vi "Complete Modern MCP Result.vi"(6 "parameters":string[][](array[string]), 7 "id in":i32, 8 "error in":errorcluster, 9 "input requests":string, 10 "handler response":string, 11 "MCP Request Metadata":T1) -> (0 "error out":errorcluster, 2 "status code":u16, 3 "response":string)   [LabVIEW 2020, in "MCP Server.lvlib"]
doc: "Turns what the request handler answered into the HTTP response body and status of a request that was not refused.\n\nLEGACY requests: the handler's answer is returned unchanged.\n\nMODERN requests (MCP 2026-07-28):\n- server/discover is answered here (supportedVersions = all versions, capabilities and serverInfo as initialize reports them, and the cache hints of Cache Hints.vi).\n- A tools/call for which a tool registered questions is answered with {\"resultType\":\"input_required\",\"inputRequests\":{...}} instead of the tool result (no requestState: the retry carries the original params with inputResponses).\n- Every other result gets \"resultType\":\"complete\" and _meta io.modelcontextprotocol/serverInfo; the methods named in Cache Hints.vi also get ttlMs and cacheScope.\n- resources/read errors -32002 (resource not found) become -32602.\n\nserverInfo is taken from initialize.vi (called with a synthetic initialize request, only for modern requests), so name and version always match what initialize reports.\n\nstatus code is 202 when there is nothing to answer (empty response to a notification), otherwise 200.\n\nThe JSONtext errors are merged and cleared here. error in is passed through unchanged and does not stop the completion."
uses:
  MCP Server.lvlib
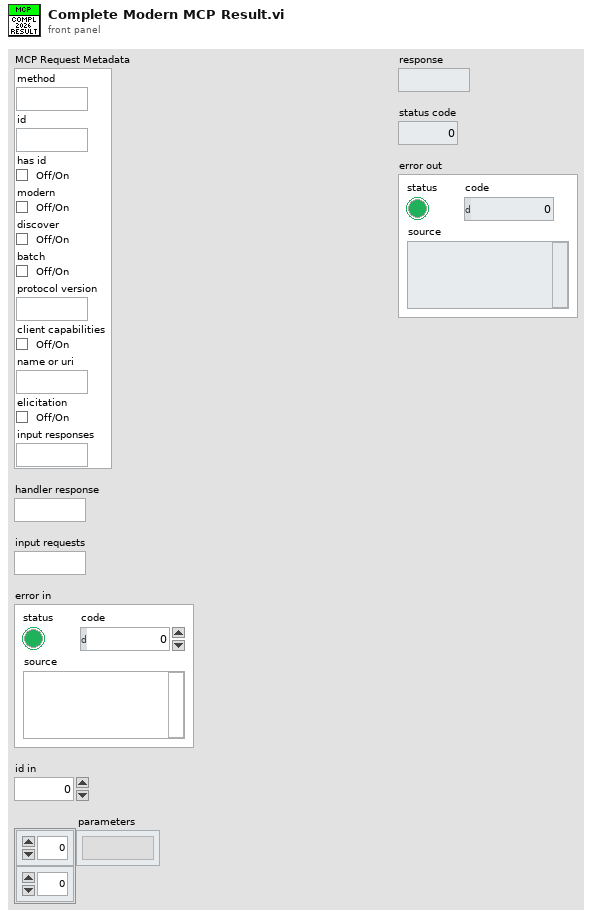
[diagram p1: front panel]
types:
  T1 = cluster{"method":string, "id":string, "has id":bool, "modern":bool, "discover":bool, "batch":bool, "protocol version":string, "client capabilities":bool, "name or uri":string, "elicitation":bool, "input responses":string}
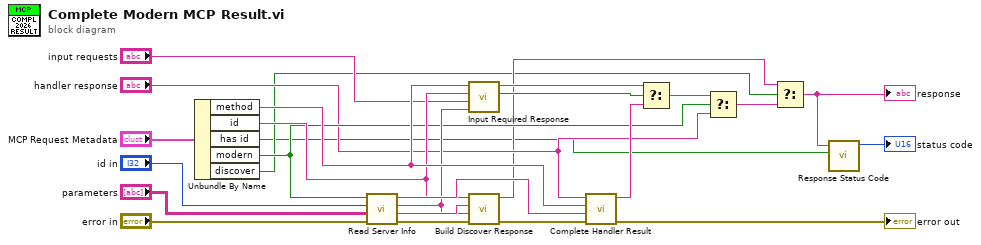
[diagram p0: block diagram]
diagram:
  n1 = Unbundle By Name("MCP Request Metadata") -> ("method"=w17:string, "id"=w16:string, "has id"=w4:bool, "modern"=w9:bool, "discover"=w6:bool)
  n2 = call "Read Server Info.vi"("error in"="error in", "parameters"="parameters", "id in"="id in", "read?"=w9) -> ("error out"=w20:errorcluster, "capabilities"=w21:string, "_meta"=w14:string, "serverInfo"=w19:string)  [unwired: 4 in]
  n3 = call "Input Required Response.vi"("_meta"=w14, "input requests"="input requests", "id"=w16, "method"=w17) -> ("input required?"=w12:bool, "response"=w13:string)  [unwired: 6 in]
  n4 = call "Build Discover Response.vi"("error in"=w20, "_meta"=w14, "capabilities"=w21, "id"=w16) -> ("error out"=w18:errorcluster, "response"=w7:string)  [unwired: 6 in]
  n5 = call "Complete Handler Result.vi"("error in"=w18, "serverInfo"=w19, "method"=w17, "handler response"="handler response") -> ("error out"=→"error out":errorcluster, "response"=w11:string)  [unwired: 6 in]
  n6 = Select(t=w13, s=w12, f=w11) -> (s? t:f=w10:string)
  n7 = Select(t=w10, s=w9, f="handler response") -> (s? t:f=w5:string)
  n8 = Select(t=w7, s=w6, f=w5) -> (s? t:f=w3:string)
  "response" <- w3
  n9 = call "Response Status Code.vi"("has id"=w4, "response"=w3) -> ("status code"=→"status code":u16)  [unwired: 9 in]
